vi "FP Snapshot Helper.vi"() -> ()   [LabVIEW 2026]
doc: "Scripting helper: saves an image of a VI's whole front panel (not only the visible area) to a PNG file."
panel:
  out "error out":errorcluster
  in  "error in":errorcluster
  in  "png path":string
  in  "vi path":string
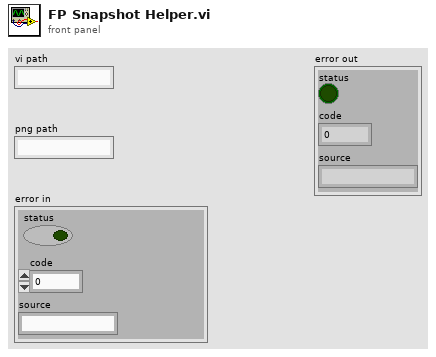
[diagram p1: front panel]
types:
  T1 = typedef "imagedata.ctl" = cluster{"image type":i32, "image depth":i32, "image":u8[], "mask":u8[], "colors":u32[], "Rectangle":cluster{"left":i16, "top":i16, "right":i16, "bottom":i16}}
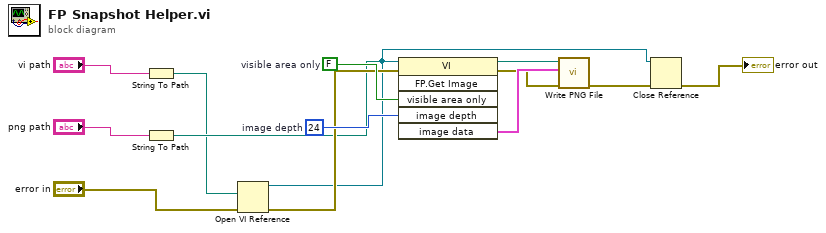
[diagram p0: block diagram]
diagram:
  w9 = 24  # image depth
  w8 = FALSE  # visible area only
  n1 = String To Path(string="vi path") -> (path=w4:path)
  n2 = String To Path(string="png path") -> (path=w5:path)
  n3 = Open VI Reference(vi path=w4, error in (no error)="error in") -> (vi reference=w6:refnum<vi>, error out=w7:errorcluster)  [unwired: 4 in]
  n4 = invoke class="VI" method="FP.Get Image"(reference=w6, error in=w7, "visible area only"=w8, "image depth"=w9) -> (error out=w10:errorcluster, "image data"=w11:T1)  [unwired: 2 in, 4 out]
  n5 = call <vilib>:"Write PNG File.vi"("error in (no error)"=w10, "image data"=w11, "path to PNG file"=w5) -> ("error out"=w12:errorcluster)  [unwired: 7 in, 1 out]
  n6 = Close Reference(reference=w6, error in (no error)=w12) -> (error out=→"error out":errorcluster)
